vi "LTE Call Process.vi"(8 "error in (no error)":errorcluster caption="에러 입력(에러 없음)", 10 "LTE Call Process Param":T1, 11 "Instrument Manager 입력":refnum<class "Instrument Manager.lvclass">) -> (0 "error out":errorcluster caption="에러 출력", 3 "Instrument Manager 출력":refnum<class "Instrument Manager.lvclass">)   [LabVIEW 2023, in "Instrument Manager.lvclass"]
uses:
  Instrument Manager.lvclass
  Type Definition/LTE Call Process Param.ctl
  Module/ANRITSU Call Box/Type Definition/LTE Supported BandWidth.ctl
  Instrument Manager.lvclass/Instrument Manager.ctl
  cc187df0-3091-4235-ad1f-e4f8c6eeadb1.vi
  Module/ANRITSU Call Box/ANRITSU Call Box.lvlib
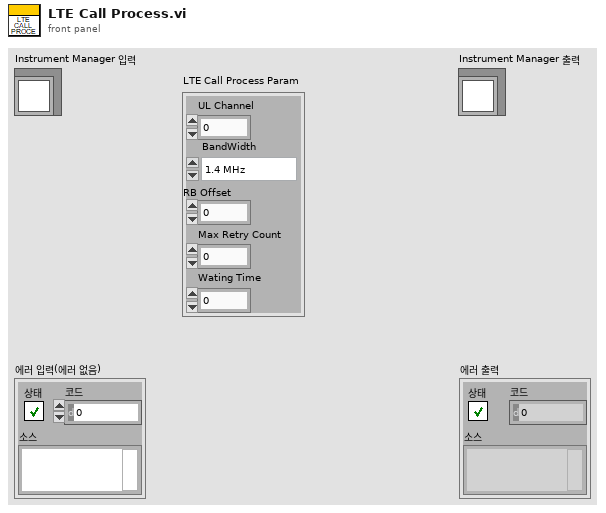
[diagram p1: front panel]
types:
  T1 = typedef "LTE Call Process Param.ctl" = cluster{"UL Channel":i32, "BandWidth":T2, "RB Offset":i32, "Max Retry Count":i32, "Wating Time":i32}
  T2 = typedef "ANRITSU Call Box.lvlib/LTE Supported BandWidth.ctl" = enum16{"1.4 MHz", "3 MHz", "5 MHz", "10 MHz", "15 MHz", "20 MHz"}
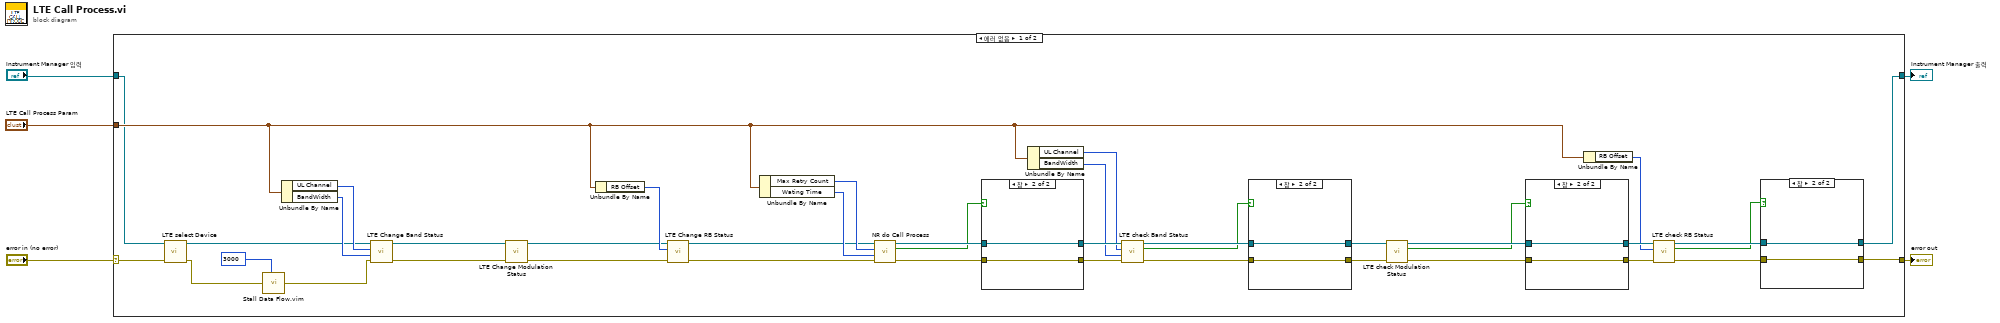
[diagram p0: block diagram]
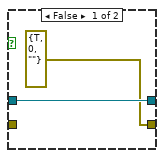
[diagram p2: hidden frame]
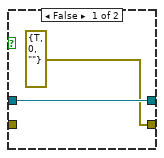
[diagram p3: hidden frame]
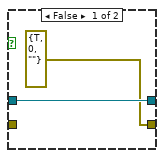
[diagram p4: hidden frame]
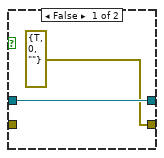
[diagram p5: hidden frame]
diagram:
  n1 = case shown="에러 없음" "error in (no error)" {
    selector: "error in (no error)" -> [w11 w64]
    tunnel: [w18 w64] -> w4
    tunnel: [w12 w63] -> w2
    tunnel: "Instrument Manager 입력" -> [w10 w63]
    tunnel: "LTE Call Process Param" -> [w14 _]
    frame No Error {
      n2 = call "LTE select Device.vi"("error in (no error)"=w11, "Instrument Manager 입력"=w10) -> ("error out"=w8:errorcluster, "Instrument Manager 출력"=w9:refnum<class "Instrument Manager.lvclass">)  [unwired: 8 in]
      n3 = call "Stall Data Flow.vim"("value in"=w8, "milliseconds to wait"=u32 3000) -> ("value out"=w7:errorcluster)  [unwired: 1 out]
      n4 = Unbundle By Name(w14) -> ("UL Channel"=w45:i32, "BandWidth"=w46:T2)
      n5 = call "LTE Change Band Status.vi"("error in (no error)"=w7, "BandWidth"=w46, "UL Channel"=w45, "Instrument Manager 입력"=w9) -> ("error out"=w44:errorcluster, "Instrument Manager 출력"=w43:refnum<class "Instrument Manager.lvclass">)  [unwired: 6 in]
      n6 = call "LTE Change Modulation Status.vi"("error in (no error)"=w44, "Instrument Manager 입력"=w43) -> ("error out"=w42:errorcluster, "Instrument Manager 출력"=w40:refnum<class "Instrument Manager.lvclass">)  [unwired: 8 in]
      n7 = Unbundle By Name(w14) -> ("RB Offset"=w41:i32)
      n8 = call "LTE Change RB Status.vi"("error in (no error)"=w42, "RB Offset"=w41, "Instrument Manager 입력"=w40) -> ("error out"=w39:errorcluster, "Instrument Manager 출력"=w36:refnum<class "Instrument Manager.lvclass">)  [unwired: 7 in]
      n9 = Unbundle By Name(w14) -> ("Max Retry Count"=w37:i32, "Wating Time"=w38:i32)
      n10 = call "NR do Call Process.vi"("error in (no error)"=w39, "Waiting Time"=w38, "Max Retry Count"=w37, "Instrument Manager 입력"=w36) -> ("error out"=w35:errorcluster, "Connected?"=w33:bool, "Instrument Manager 출력"=w34:refnum<class "Instrument Manager.lvclass">)  [unwired: 5 in]
      n11 = case shown="참" w33 {
        tunnel: w34 -> [w60 w62]
        tunnel: [w60 w62] -> w22
        tunnel: [errorcluster {"status"=TRUE, "code"=0, "source"=""} ("error out") w61] -> w24
        tunnel: w35 -> [_ w61]
        frame False {
        }
        frame True {
        }
      }
      n12 = Unbundle By Name(w14) -> ("UL Channel"=w16:i32, "BandWidth"=w17:T2)
      n13 = call "LTE check Band Status.vi"("error in (no error)"=w24, "BandWidth"=w17, "UL Channel"=w16, "Instrument Manager 입력"=w22) -> ("error out"=w23:errorcluster, "불리언"=w15:bool, "Instrument Manager 출력"=w21:refnum<class "Instrument Manager.lvclass">)  [unwired: 5 in]
      n14 = case shown="참" w15 {
        tunnel: w21 -> [w48 w50]
        tunnel: [w48 w50] -> w19
        tunnel: [errorcluster {"status"=TRUE, "code"=0, "source"=""} ("error out") w49] -> w20
        tunnel: w23 -> [_ w49]
        frame False {
        }
        frame True {
        }
      }
      n15 = call "LTE check Modulation Status.vi"("error in (no error)"=w20, "Instrument Manager 입력"=w19) -> ("error out"=w32:errorcluster, "불리언"=w30:bool, "Instrument Manager 출력"=w31:refnum<class "Instrument Manager.lvclass">)  [unwired: 7 in]
      n16 = case shown="참" w30 {
        tunnel: w31 -> [w56 w58]
        tunnel: [w56 w58] -> w28
        tunnel: [errorcluster {"status"=TRUE, "code"=0, "source"=""} ("error out") w57] -> w29
        tunnel: w32 -> [_ w57]
        frame False {
        }
        frame True {
        }
      }
      n17 = Unbundle By Name(w14) -> ("RB Offset"=w13:i32)
      n18 = call "LTE check RB Status.vi"("error in (no error)"=w29, "RB Offset"=w13, "Instrument Manager 입력"=w28) -> ("error out"=w27:errorcluster, "불리언"=w25:bool, "Instrument Manager 출력"=w26:refnum<class "Instrument Manager.lvclass">)  [unwired: 6 in]
      n19 = case shown="참" w25 {
        tunnel: w26 -> [w52 w54]
        tunnel: [w52 w54] -> w12
        tunnel: [errorcluster {"status"=TRUE, "code"=0, "source"=""} ("error out") w53] -> w18
        tunnel: w27 -> [_ w53]
        frame False {
        }
        frame True {
        }
      }
    }
    frame Error {
    }
  }
  "error out" <- w4
  "Instrument Manager 출력" <- w2
